vi "user32 GetWindow.vi"(0 "hWnd":u64, 5 "uCmd":u32=4, 11 "error in":errorcluster) -> (4 "window":u64, 15 "error out":errorcluster)   [LabVIEW 2020, in "RemoteVI.lvlib"]
doc: "Returns a window related to hWnd through user32.dll GetWindow (stdcall, called in any thread). uCmd 4 GW_OWNER (default) gives the OWNER of a top-level window - the window it stays in front of and is hidden with; 0 when it has none. Other values: 0 GW_HWNDFIRST, 1 GW_HWNDLAST, 2 GW_HWNDNEXT, 3 GW_HWNDPREV, 5 GW_CHILD, 6 GW_ENABLEDPOPUP. window is 0 when there is no such window. When error in carries an error the DLL is not called. Generated by scripts\\Build Win32 Wrappers.vi - do not edit by hand, rebuild it."
uses:
  RemoteVI.lvlib
  user32.dll
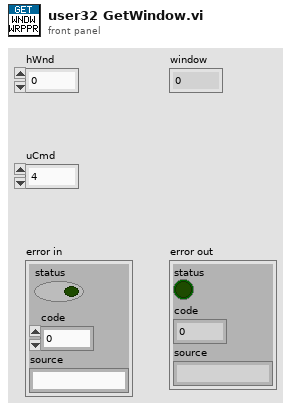
[diagram p1: front panel]
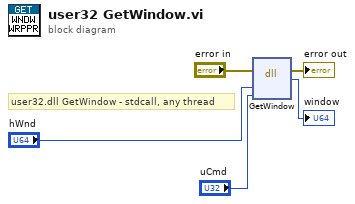
[diagram p0: block diagram]
diagram:
  # "user32.dll GetWindow - stdcall, any thread"
  n1 = dll-call lib="user32.dll" fn="GetWindow"(error in="error in", "hWnd"="hWnd", "uCmd"="uCmd") -> (error out=→"error out":errorcluster, →"window":u64)  [unwired: 4 in, 1 out]
